vi "FuncVI-MADev.vi"(5 "InstanceRef":T2, 9 "arg list":T1[](array[typedef]) {"num" format="%.2f"}) -> (0 "error out":bool, 3 "result":T1 {"num" format="%.2f"})   [LabVIEW 2021]
doc: "::: CalcExpress Toolkit :::\nCopyright (c) 2000-2026 Konstantin Shifershteyn. All rights reserved."
uses:
  cetypes.llb/CalcExpress Function Argument Info.ctl
  cetypes.llb/CalcExpress Instance RefNum.ctl
  <vilib>/Analysis/baseanly.llb/Mean (DBL).vi
  <vilib>/Analysis/NI_AALBase.lvlib
panel:
  in  "max arg num":i32=1
  in  "min arg num":i32=1
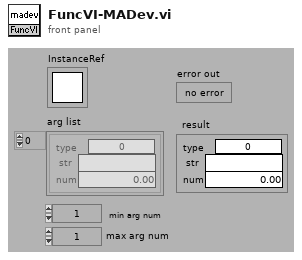
[diagram p1: front panel]
types:
  T1 = typedef "CalcExpress Function Argument Info.ctl" = cluster{"type":u32, "str":string, "num":dbl}
  T2 = typedef "CalcExpress Instance RefNum.ctl" = refnum<k1>
  T3 = enum32{"String", "DBL Number", "identifier", "1D Array of DBL", "2D Array of DBL", "CDB Number", "1D Array of CDB", "2D Array of CDB", "1D Array of String", "2D Array of String", "Unknown data type"}
  T4 = cluster{"use this constant to specify a predefined type":enum32{"String", "DBL Number", "identifier", "1D Array of DBL", "2D Array of DBL", "CDB Number", "1D Array of CDB", "2D Array of CDB", "1D Array of String", "2D Array of String", "Unknown data type"}, string, dbl}
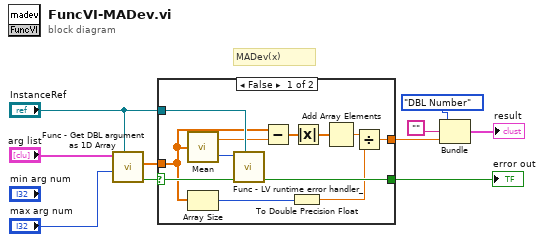
[diagram p0: block diagram]
diagram:
  # "MADev(x)"
  n1 = call "Func - Get DBL argument as 1D Array.vi"("InstanceRef"="InstanceRef", "max arg num"="max arg num", "arg list"="arg list") -> ("error out"=w10:bool, "1D data"=w9:dbl[])  [unwired: 5 in, 2 out]
  n2 = case shown="False" w10 {
    selector: w10 -> [w22 w23]
    tunnel: w9 -> [w17 _]
    tunnel: [w12 _] -> w2
    tunnel: [w20 w23] -> w6
    tunnel: "InstanceRef" -> [w19 _]
    frame False {
      n3 = call-poly <vilib>:"Mean.vi"("X"=w17) -> ("mean"=w18:dbl, "error"=w21:i32)
      n4 = Array Size(array=w17) -> (size(s)=w16:i32)
      n5 = call "Func - LV runtime error handler_.vi"("InstanceRef"=w19, "error in"=w22, "LabVIEW error code"=w21) -> ("error out"=w20:bool)  [unwired: 8 in]
      n6 = Subtract(x=w17, y=w18) -> (x-y=w15:dbl[])
      n7 = To Double Precision Float(number=w16) -> (double precision float=w11:dbl)
      n8 = Absolute Value(x=w15) -> (abs(x)=w14:dbl[])
      n9 = Add Array Elements(numeric array=w14) -> (sum=w13:dbl)
      n10 = Divide(x=w13, y=w11) -> (x/y=w12:dbl)
    }
    frame True {
    }
  }
  "error out" <- w6
  n11 = Bundle("use this constant to specify a predefined type"=T3."DBL Number", "", w2) -> (→"result":T4)  [unwired: 1 in]
